vi "Cleanup VI BD.vi"(8 "error in (no error)":errorcluster, 11 "VI in":refnum<vi>) -> (0 "error out":errorcluster, 3 "VI out":refnum<vi>)   [LabVIEW 2019, in "gRPC Template Creation Utility.lvlib"]
uses:
  gRPC Template Creation Utility.lvlib
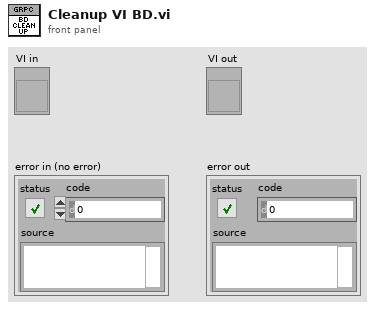
[diagram p1: front panel]
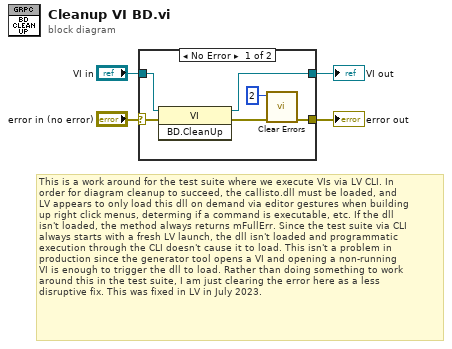
[diagram p0: block diagram]
diagram:
  # "This is a work around for the test suite where we execute VIs via LV CLI. In\norder for diagram cleanup to succeed, the callisto.dll must be loaded, and\nLV appears to only load this dll on demand via editor gestures when building\nup right click menus, determing if a command is executable, etc. If the dll\nisn't loaded, the method always returns mFullErr. Since the test suite via CLI\nalways starts with a fresh LV launch, the dll isn't loaded and programmatic\nexecution through the CLI doesn't cause it to load. This isn't a problem in\nproduction since the generator tool opens a VI and opening a non-running\nVI is enough to trigger the dll to load. Rather than doing something to work\naround this in the test suite, I am just clearing the error here as a less \ndisruptive fix. This was fixed in LV in July 2023."
  n1 = case shown="No Error" "error in (no error)" {
    selector: "error in (no error)" -> [w8 w11]
    tunnel: [w6 w11] -> w4
    tunnel: [w10 w12] -> w3
    tunnel: "VI in" -> [w9 w12]
    frame No Error {
      n2 = invoke class="VI" method="BD.CleanUp"(reference=w9, error in=w8) -> (reference out=w10:refnum<vi>, error out=w7:errorcluster)  [unwired: 1 in, 1 out]
      n3 = call <vilib>:"Clear Errors.vi"("error in (no error)"=w7, "specific error code to clear (0: all)"=2) -> ("error out"=w6:errorcluster)  [unwired: 4 in, 1 out]
    }
    frame Error {
    }
  }
  "error out" <- w4
  "VI out" <- w3
